vi "test resource templates list.vi"(8 "error in (no error)":errorcluster) -> (0 "error out":errorcluster, 3 "body":string)   [LabVIEW 2020, in "MCP Server tests.lvlib"]
doc: "resources/templates/list must be answered with a resourceTemplates array (empty, this server has no templates)."
uses:
  MCP Server tests.lvlib
  <vilib>/JDP Science/JSONtext/Next JSON Value.vi
  <vilib>/JDP Science/JSONtext/String Subset.vi
  <vilib>/JDP Science/JSONtext/Parsing/Advance past next JSON Value (inlined COPY).vi
  <vilib>/JDP Science/JSONtext/Parsing/Advance past whitespace.vi
  <vilib>/JDP Science/JSONtext/Parsing/Advance past String.vi
  <vilib>/JDP Science/JSONtext/Parsing/Advance past Number.vi
  <vilib>/JDP Science/JSONtext/Parsing/Advance past Line Ending.vi
  <vilib>/JDP Science/JSONtext/Parsing/Parse Full Path or Item Name.vi
  <vilib>/JDP Science/JSONtext/Parsing/Advance past Array.vi
  <vilib>/JDP Science/JSONtext/Parsing/Advance past Object.vi
  <vilib>/JDP Science/JSONtext/support/Error Cluster From Code.vi
  <vilib>/JDP Science/JSONtext/Offset/Find Item Locations by Path.vi
  <vilib>/addons/_JKI Toolkits/Caraya/classes/Test/Test.lvclass
  <vilib>/JDP Science/JSONtext/JSONtext.lvlib
  <vilib>/addons/_JKI Toolkits/Caraya/classes/Assert/Assert.lvclass
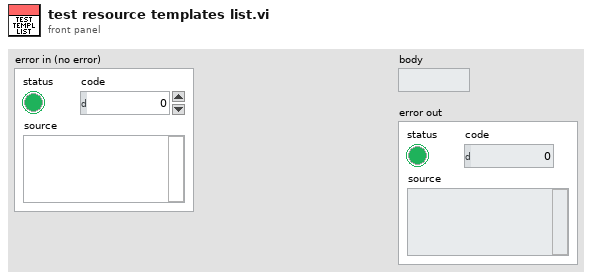
[diagram p1: front panel]
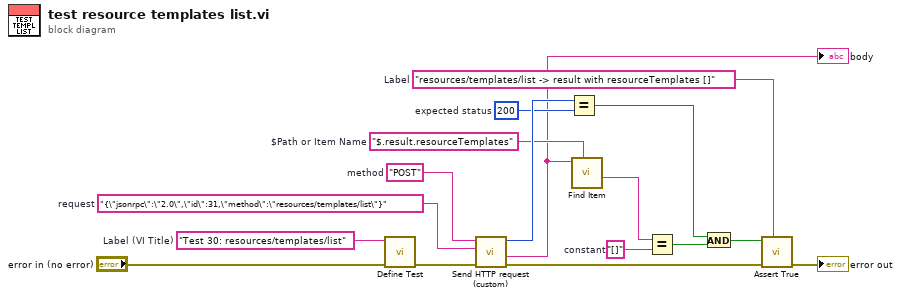
[diagram p0: block diagram]
diagram:
  w3 = "resources/templates/list -> result with resourceTemplates []"  # Label
  w8 = "[]"  # constant
  w10 = "$.result.resourceTemplates"  # $Path or Item Name
  w11 = 200  # expected status
  w14 = "{\"jsonrpc\":\"2.0\",\"id\":31,\"method\":\"resources/templates/list\"}"  # request
  w15 = "POST"  # method
  w17 = "Test 30: resources/templates/list"  # Label (VI Title)
  n1 = call <vilib>:"Define Test.vi"("error in (no error)"="error in (no error)", "Label (VI Title)"=w17) -> ("error out"=w13:errorcluster)  [unwired: 8 in, 1 out]
  n2 = call "Send HTTP request (custom).vi"("error in (no error)"=w13, "request"=w14, "method"=w15) -> ("error out"=w4:errorcluster, "response"=w2:string, "status code"=w12:i32)  [unwired: 5 in, 1 out]
  "body" <- w2
  n3 = Equal?(x=w12, y=w11) -> (x = y?=w7:bool)
  n4 = call <vilib>:"Find Item.vi"("$Path or Item Name"=w10, "JSON"=w2) -> ("<JSON>"=w9:string)  [unwired: 6 in, 3 out]
  n5 = Equal?(x=w9, y=w8) -> (x = y?=w6:bool)
  n6 = And(x=w7, y=w6) -> (x .and. y?=w5:bool)
  n7 = call <vilib>:"Assert True.vi"("Label"=w3, "error in (no error)"=w4, "True?"=w5) -> ("error out"=→"error out":errorcluster)  [unwired: 7 in, 1 out]
